vi "Set-Clear GPIO.vi"   [LabVIEW 2020, in "wiringPi.lvlib"]
doc: "<b>_______________________________________________________________</b>\n** Author: Juan José Villacorta\n** LabVIEW wrapper for C library <b> wiringPi </b>,\n** https://github.com/WiringPi/WiringPi\n<b>_______________________________________________________________</b>\n\n/*\n * digitalWrite:\n * Set an output bit\n *********************************************************************************\n */"
uses:
  wiringPi.lvlib
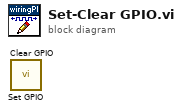
[diagram p0: block diagram]
diagram:
  n1 = call "Set GPIO.vi"() -> ()  [unwired: 10 in, 2 out]
  n2 = call "Clear GPIO.vi"() -> ()  [unwired: 10 in, 2 out]
